vi "session_callback.vi"() -> ()   [LabVIEW 2017]
doc: "Illustrates how to register for session callback events."
uses:
  libssh2/libssh2_session_callback_type.ctl
  libssh2/libssh2_session_abstract.ctl
  libssh2/libssh2_session_handshake_tcp.vi
  libssh2/libssh2_init_default.vi
  <vilib>/Utility/tcp.llb/TCP Get Raw Net Object.vi
  libssh2/libssh2_session_handshake_socket.vi
  libssh2/libssh2_userauth_password_ex.vi
  libssh2/libssh2_channel_open_ex.vi
  libssh2/libssh2_channel_process_startup.vi
  libssh2/libssh2_channel_read_ex.vi
  libssh2/libssh2.lvlib
panel:
  out "Output":string
  out "exitsignal":string
  out "exit status":i32
  in  "command":string="ping localhost -c 1"
  in  "password":string
  in  "username":string
  out "error out":errorcluster
  in  "hostname":string="localhost"
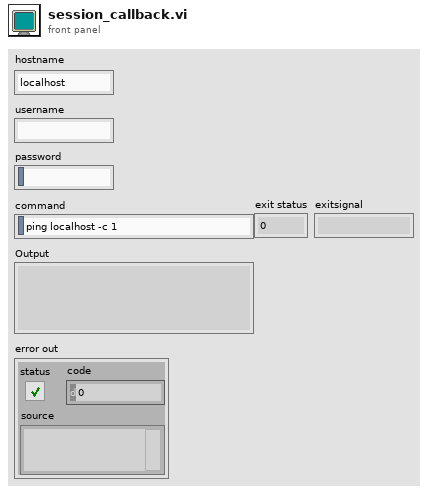
[diagram p1: front panel]
types:
  T1 = typedef "libssh2.lvlib/libssh2_session_abstract.ctl" = cluster{"send":refnum<vi>, "receive":refnum<vi>, "keyboard-interactive response":refnum<vi>}
  T2 = typedef "libssh2.lvlib/libssh2_session_callback_type.ctl" = enum16{"Ignore", "Debug", "Disconnect", "MAC Error", "X11", "Send", "Receive", "Auth Agent", "Auth Agent Identities", "Auth Agent Sign"}
  T3 = typedef "libssh2.lvlib/Session Refnum.ctl" = refnum<k1>
  T4 = typedef "libssh2.lvlib/Channel Refnum.ctl" = refnum<k1>
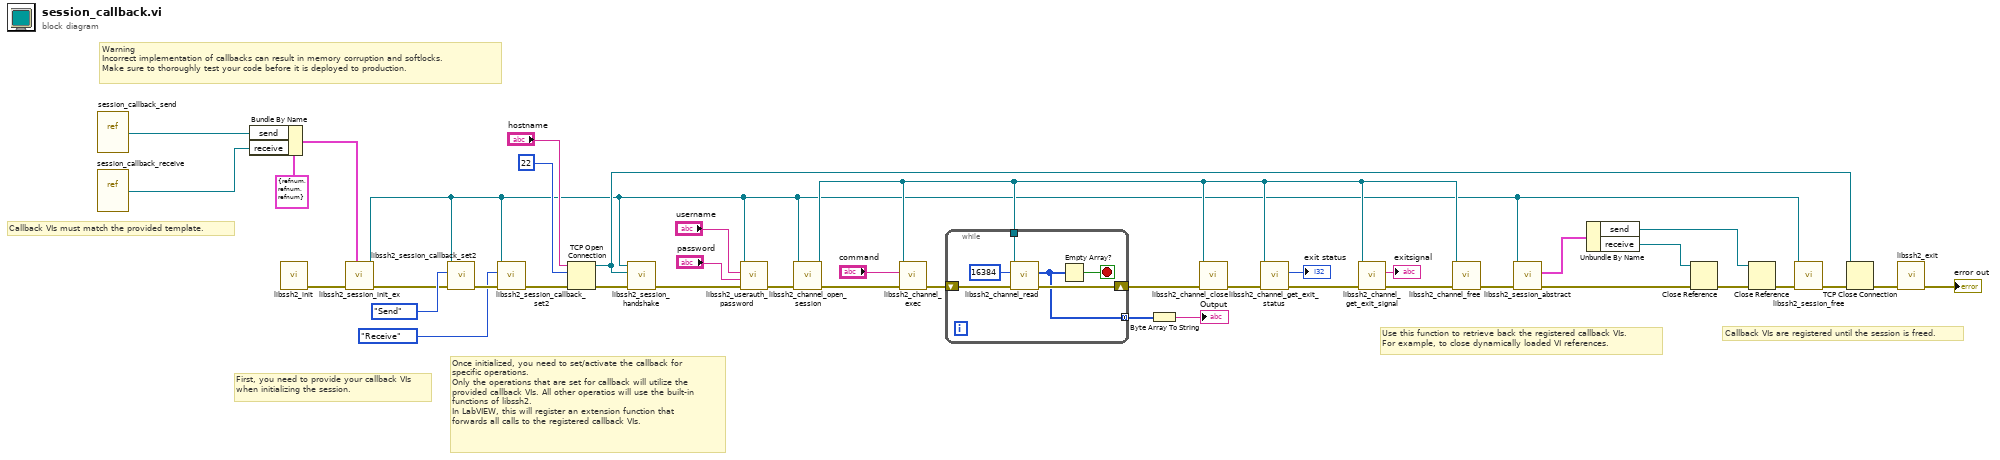
[diagram p0: block diagram]
diagram:
  # "Use this function to retrieve back the registered callback VIs.\nFor example, to close dynamically loaded VI references."
  # "Callback VIs are registered until the session is freed."
  # "Warning\nIncorrect implementation of callbacks can result in memory corruption and softlocks.\nMake sure to thoroughly test your code before it is deployed to production."
  # "Callback VIs must match the provided template."
  # "Once initialized, you need to set/activate the callback for specific operations.\nOnly the operations that are set for callback will utilize the provided callback VIs. All other operatios will use the built-in functions of libssh2.\nIn LabVIEW, this will register an extension function that forwards all calls to the registered callback VIs."
  # "First, you need to provide your callback VIs when initializing the session."
  n1 = vi-ref "session_callback_send.vi"() -> (w12:refnum<vi>)
  n2 = vi-ref "session_callback_receive.vi"() -> (w10:refnum<vi>)
  n3 = Bundle By Name(cluster=T1 {"send"=refnum, "receive"=refnum, "keyboard-interactive response"=refnum} ("abstract"), "send"=w12, "receive"=w10) -> (w11:T1)
  n4 = call-poly "libssh2_init.vi"() -> ("error out"=w41:errorcluster)  [unwired: 11 in]
  n5 = call "libssh2_session_init_ex.vi"("abstract"=w11, "error in (no error)"=w41) -> ("error out"=w9:errorcluster, "session"=w7:T3)  [unwired: 8 in]
  n6 = call "libssh2_session_callback_set2.vi"("error in (no error)"=w9, "callback type"=libssh2_session_callback_type."Send", "session"=w7) -> ("error out"=w16:errorcluster)  [unwired: 7 in, 1 out]
  n7 = call "libssh2_session_callback_set2.vi"("error in (no error)"=w16, "callback type"=libssh2_session_callback_type."Receive", "session"=w7) -> ("error out"=w15:errorcluster)  [unwired: 7 in, 1 out]
  n8 = TCP Open Connection(address="hostname", remote port or service name=u16 22, error in (no error)=w15) -> (connection ID=w20:refnum<k5>, error out=w21:errorcluster)  [unwired: 2 in]
  n9 = call-poly "libssh2_session_handshake.vi"("error in (no error)"=w21, "tcp connection"=w20, "session"=w7) -> ("error out"=w19:errorcluster)  [unwired: 8 in]
  n10 = call "libssh2_userauth_password.vi"("error in (no error)"=w19, "password"="password", "username"="username", "session"=w7) -> ("error out"=w37:errorcluster)  [unwired: 7 in]
  n11 = call "libssh2_channel_open_session.vi"("error in (no error)"=w37, "session"=w7) -> ("error out"=w34:errorcluster, "channel"=w27:T4)  [unwired: 8 in]
  n12 = call "libssh2_channel_exec.vi"("error in (no error)"=w34, "command"="command", "channel"=w27) -> ("error out"=w33:errorcluster)  [unwired: 8 in]
  n13 = while {
    tunnel: w27 -> [w44]
    tunnel: [w42] -> w25 mode=concatenating
    shift-right: [w46] -> w31
    shift-left: w33 -> [w47]
    stop <- w43 stop-if-true
    n14 = call "libssh2_channel_read.vi"("error in (no error)"=w47, "buffer length"=16384 ("buflen"), "channel"=w44) -> ("error out"=w46:errorcluster, "buffer"=w42:u8[])  [unwired: 7 in]
    n15 = Empty Array?(array=w42) -> (empty?=w43:bool)
  }
  n16 = Byte Array To String(unsigned byte array=w25) -> (string=→"Output":string)
  n17 = call "libssh2_channel_close.vi"("error in (no error)"=w31, "channel"=w27) -> ("error out"=w30:errorcluster)  [unwired: 9 in]
  n18 = call "libssh2_channel_get_exit_status.vi"("error in (no error)"=w30, "channel"=w27) -> ("error out"=w29:errorcluster, "exit status"=→"exit status":i32)  [unwired: 8 in]
  n19 = call "libssh2_channel_get_exit_signal.vi"("error in (no error)"=w29, "channel"=w27) -> ("error out"=w28:errorcluster, "exitsignal"=→"exitsignal":string)  [unwired: 6 in, 2 out]
  n20 = call "libssh2_channel_free.vi"("error in (no error)"=w28, "channel"=w27) -> ("error out"=w8:errorcluster)  [unwired: 9 in]
  n21 = call "libssh2_session_abstract.vi"("error in (no error)"=w8, "session"=w7) -> ("error out"=w4:errorcluster, "abstract"=w6:T1)  [unwired: 8 in]
  n22 = Unbundle By Name(w6) -> ("send"=w1:refnum<vi>, "receive"=w5:refnum<vi>)
  n23 = Close Reference(reference=w5, error in (no error)=w4) -> (error out=w3:errorcluster)
  n24 = Close Reference(reference=w1, error in (no error)=w3) -> (error out=w2:errorcluster)
  n25 = call "libssh2_session_free.vi"("error in (no error)"=w2, "session"=w7) -> ("error out"=w40:errorcluster)  [unwired: 9 in]
  n26 = TCP Close Connection(connection ID=w20, error in (no error)=w40) -> (error out=w23:errorcluster)  [unwired: 1 in, 1 out]
  n27 = call "libssh2_exit.vi"("error in (no error)"=w23) -> ("error out"=→"error out":errorcluster)  [unwired: 10 in]
